vi "Stages Messenger.vi"(0 "Stage Notifier Name":string="ProScan3", 2 "Actions":T2, 5 "Setpoint":dbl[](array[numeric]), 7 "Axis":bool[](array[boolean]), 9 "Velocity":dbl, 11 "Misc":variant, 12 "Servo On?":bool, 13 "Exit While Busy?":bool) -> (4 "Stage Notifier Name (Dup)":string, 6 "Positions":dbl[](array[numeric]), 8 "Status":T1, 10 "Servo Status":bool, 15 "Error":errorcluster)   [LabVIEW 2021]
uses:
  Stages Controls/Stage Actions.ctl
  Stages Controls/Stage Status.ctl
  Stages Controls/Stage Notifier Element.ctl
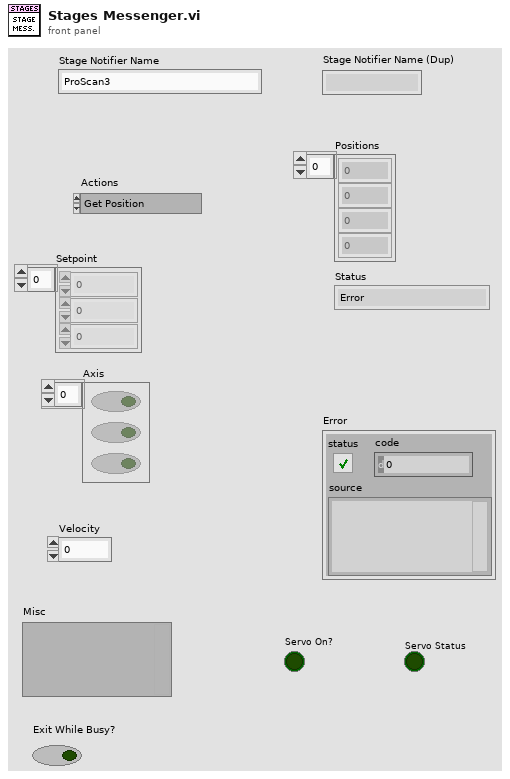
[diagram p1: front panel]
types:
  T1 = typedef "Stage Status.ctl" = enum16{"Error", "Abort", "Busy", "On Target"}
  T2 = typedef "Stage Actions.ctl" = enum16{"Get Position", "SERVO OFF", "SERVO ON", "SERVO ON/OFF", "MVR", "MOVE", "HALT", "ONTARGET", "ERROR", "REFERENCE", "INIT", "VELOCITY", "STATUS", "EXIT", "HOME", "ZEROPOS", "NANOPOS", "ANALOG", "QUIT"}
  T3 = typedef "Stage Notifier Element.ctl" = cluster{"Action":T2, "Axis":bool[], "Setpoint":dbl[], "Velocity":dbl, "Cmd Recvd?":bool, "Position":dbl[], "Status":T1, "Misc":variant, "Servo On?":bool}
  T4 = typedef "Stage Limits.ctl" = cluster{"Notifier":string, "Use Limits":bool, "Limits":dbl[][]}
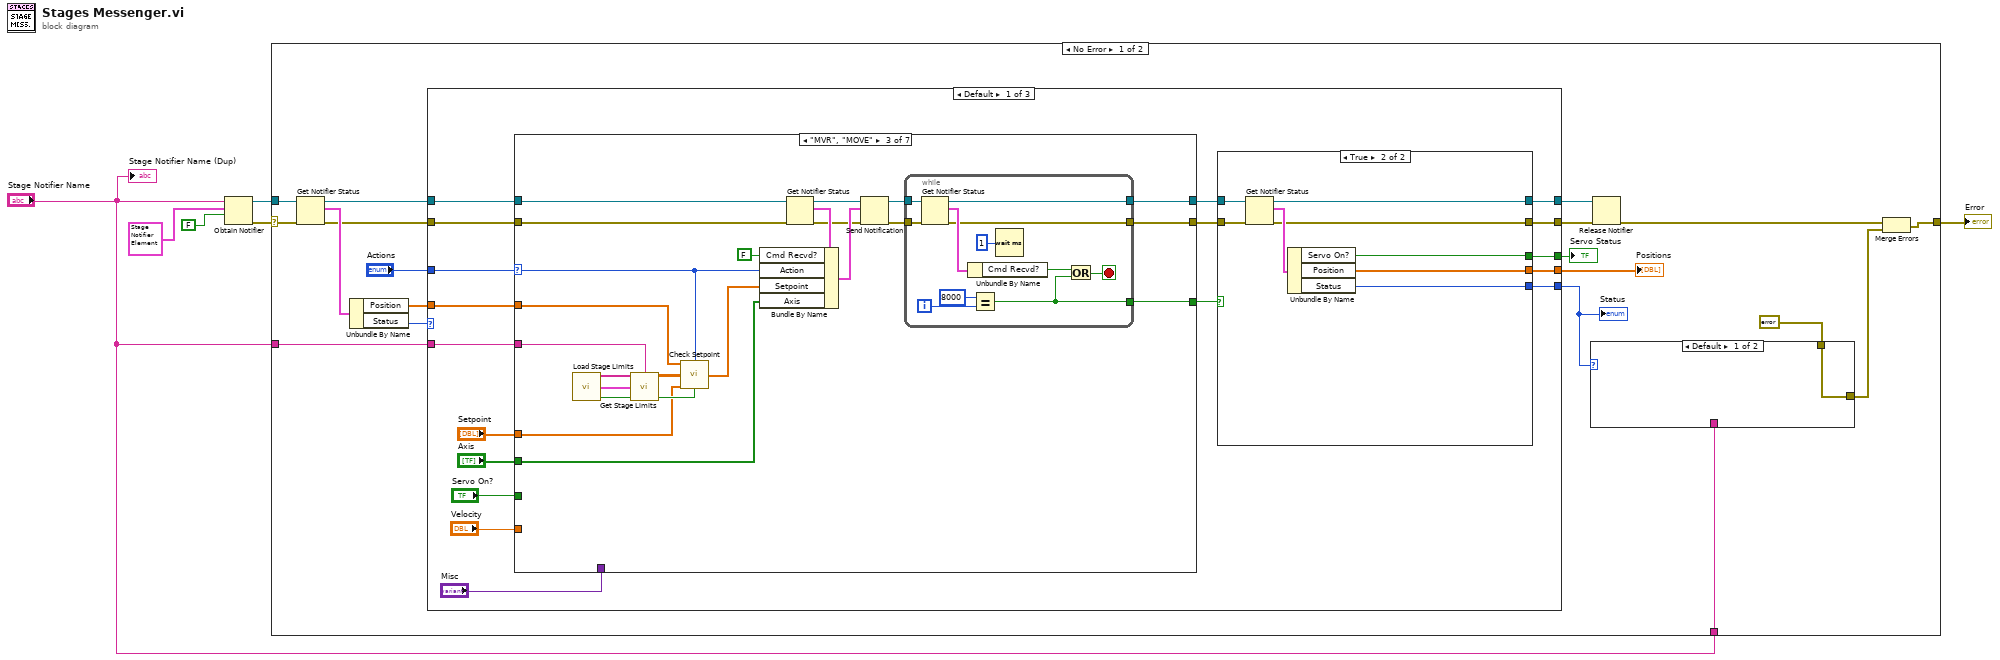
[diagram p0: block diagram]
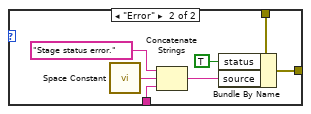
[diagram p2: hidden frame]
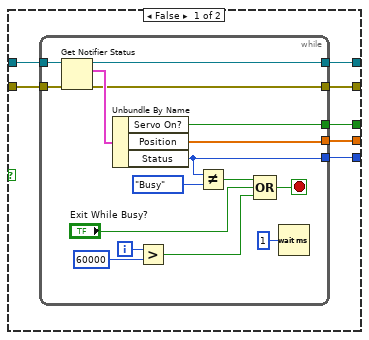
[diagram p3: hidden frame]
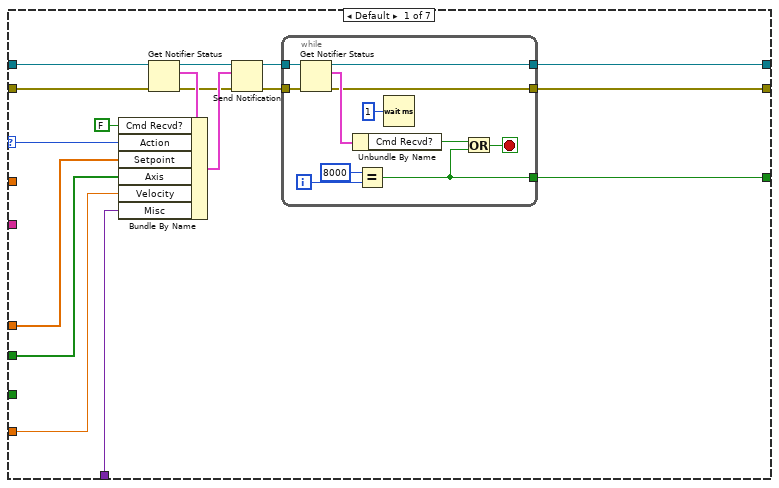
[diagram p4: hidden frame]
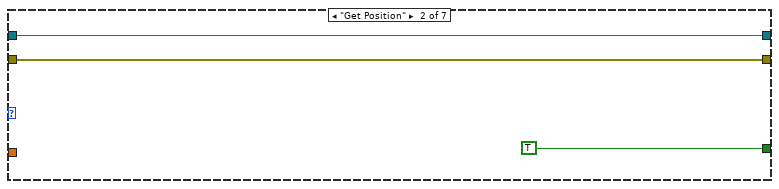
[diagram p5: hidden frame]
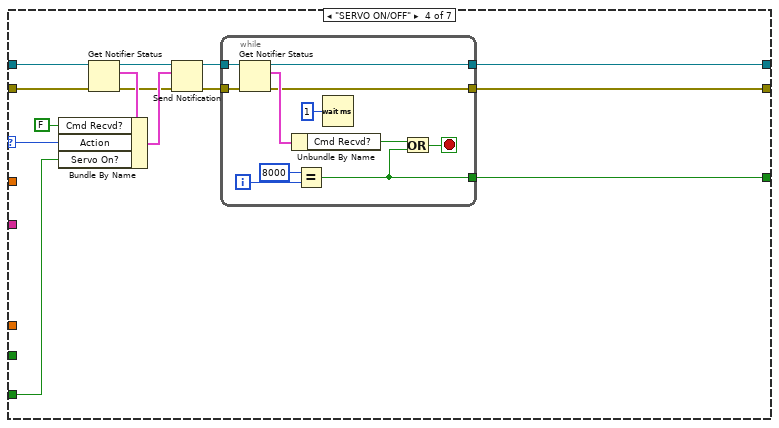
[diagram p6: hidden frame]
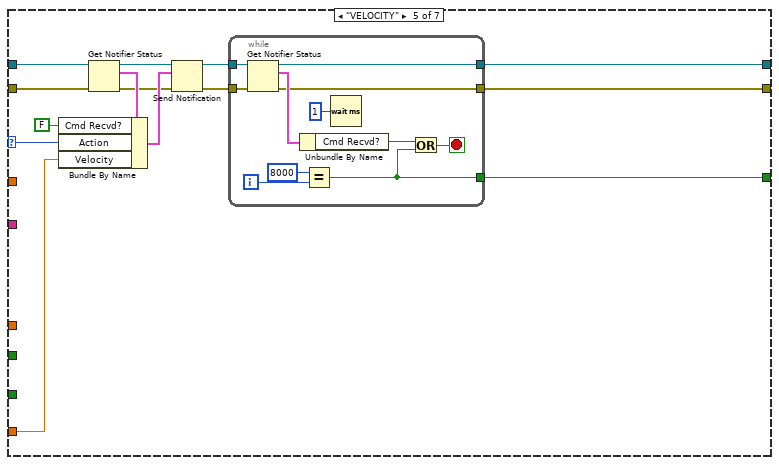
[diagram p7: hidden frame]
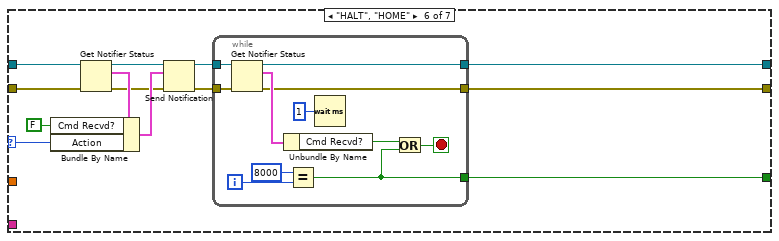
[diagram p8: hidden frame]
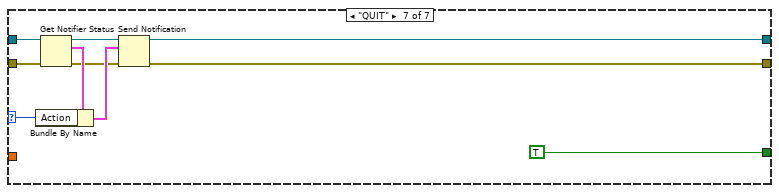
[diagram p9: hidden frame]
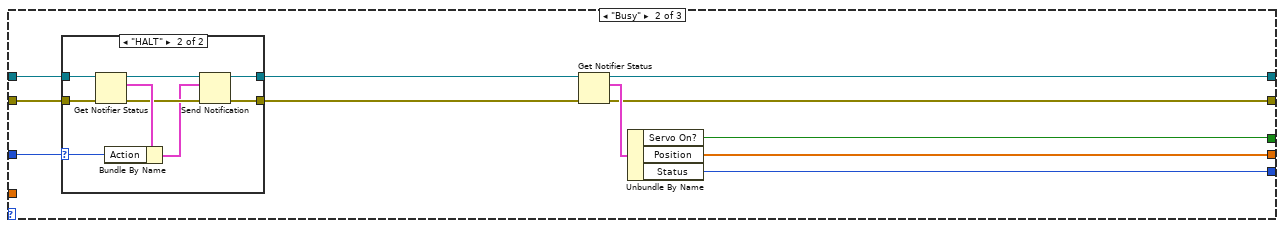
[diagram p10: hidden frame]
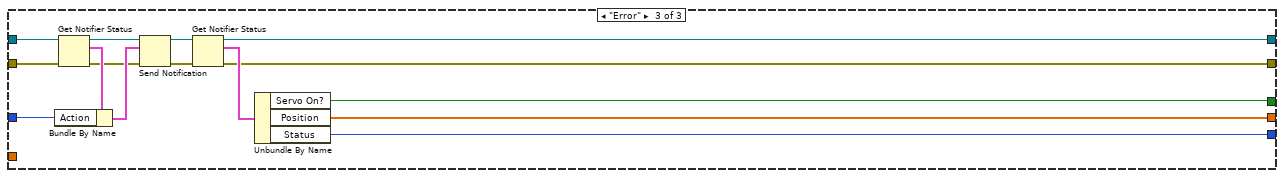
[diagram p12: hidden frame]
diagram:
  n1 = Obtain Notifier(name (unnamed)="Stage Notifier Name", notification data type=T3 {"Action"=enum."Get Position", "Axis"=[], "Setpoint"=[], "Velocity"=0.5, "Cmd Recvd?"=FALSE, "Position"=[], "Status"=enum."Error", "Misc"=variant, "Servo On?"=FALSE} ("Stage Status"), create if not found? (T)=FALSE) -> (notifier out=w3:refnum<notifier>, error out=w4:errorcluster)  [unwired: 1 in, 1 out]
  n2 = case shown="No Error" w4 {
    selector: w4 -> [w19 w269]
    tunnel: w3 -> [w25 _]
    tunnel: "Stage Notifier Name" -> [w14 _]
    tunnel: [w11 w269] -> w2
    tunnel: "Stage Notifier Name" -> [w7 _]
    frame No Error {
      n3 = Get Notifier Status(notifier=w25, error in (no error)=w19) -> (notifier out=w23:refnum<notifier>, current notification=w24:T3, error out=w18:errorcluster)  [unwired: 2 out]
      n4 = Unbundle By Name(w24) -> ("Position"=w8:dbl[], "Status"=w16:T1)
      n5 = case shown="Default" w16 {
        tunnel: w23 -> [w51 w236 w268]
        tunnel: [w44 w241 w262] -> w22
        tunnel: [w43 w240 w261] -> w21
        tunnel: [w42 w239 w260] -> w15
        tunnel: "Actions" -> [w50 w237 w266]
        tunnel: w18 -> [w41 w235 w258]
        tunnel: [w39 w238 w255] -> w17
        tunnel: [w36 w232 w254] -> w9
        tunnel: w8 -> [w35 _ _]
        tunnel: w7 -> [w34 _ _]
        frame Default {
          n6 = case shown="\"MVR\", \"MOVE\"" w50 {
            selector: w50 -> [w95 _ w119 w157 w182 w206 w227]
            tunnel: w51 -> [w96 w113 w133 w158 w183 w207 w230]
            tunnel: [w88 w113 w130 w154 w179 w203 w231] -> w45
            tunnel: "Setpoint" -> [w92 _ w116 _ _ _ _]
            tunnel: "Axis" -> [w91 _ w115 _ _ _ _]
            tunnel: "Velocity" -> [w90 _ _ _ w173 _ _]
            tunnel: "Misc" -> [w89 _ _ _ _ _ _]
            tunnel: [w87 TRUE w129 w153 w178 w202 TRUE] -> w46
            tunnel: w41 -> [w86 w112 w128 w152 w177 w201 w224]
            tunnel: [w83 w112 w125 w149 w174 w198 w222] -> w40
            tunnel: "Servo On?" -> [_ _ _ w148 _ _ _]
            tunnel: w35 -> [_ _ w118 _ _ _ _]
            tunnel: w34 -> [_ _ w117 _ _ _ _]
            frame Default {
              n7 = Get Notifier Status(notifier=w96, error in (no error)=w86) -> (notifier out=w97:refnum<notifier>, current notification=w98:T3, error out=w85:errorcluster)  [unwired: 2 out]
              n8 = Bundle By Name(cluster=w98, "Cmd Recvd?"=FALSE, "Action"=w95, "Setpoint"=w92, "Axis"=w91, "Velocity"=w90, "Misc"=w89) -> (w99:T3)
              n9 = Send Notification(notification=w99, notifier=w97, error in (no error)=w85) -> (notifier out=w93:refnum<notifier>, error out=w84:errorcluster)
              n10 = while {
                tunnel: w93 -> [w110]
                tunnel: [w107] -> w88
                tunnel: [w103] -> w87
                tunnel: w84 -> [w101]
                tunnel: [w100] -> w83
                i -> [w106]
                stop <- w102 stop-if-true
                n11 = Get Notifier Status(notifier=w110, error in (no error)=w101) -> (notifier out=w107:refnum<notifier>, current notification=w109:T3, error out=w100:errorcluster)  [unwired: 2 out]
                n12 = Unbundle By Name(w109) -> ("Cmd Recvd?"=w104:bool)
                n13 = Equal?(x=8000, y=w106) -> (x = y?=w103:bool)
                n14 = Wait (ms)(milliseconds to wait=u32 1) -> ()  [unwired: 1 out]
                n15 = Or(x=w104, y=w103) -> (x .or. y?=w102:bool)
              }
            }
            frame "Get Position" {
            }
            frame "MVR", "MOVE" {
              n16 = call "Load Stage Limits.vi"() -> ("Notifier Names"=w122:string[], "Stage Limits"=w123:T4[], "Loaded"=w124:bool)  [unwired: 13 in]
              n17 = call "Get Stage Limits.vi"("Notifier Names"=w122, "Notifier Name"=w117, "Stage Limits"=w123, "Limits Loaded?"=w124) -> ("Limits"=w120:dbl[][], "Use Limits?"=w121:bool)  [unwired: 10 in]
              n18 = call "Check Setpoint.vi"("Positions"=w118, "Actions"=w119, "Limits"=w120, "Setpoints"=w116, "Use Limits"=w121) -> ("Setpoints Out"=w114:dbl[])  [unwired: 10 in]
              n19 = Get Notifier Status(notifier=w133, error in (no error)=w128) -> (notifier out=w134:refnum<notifier>, current notification=w135:T3, error out=w127:errorcluster)  [unwired: 2 out]
              n20 = Bundle By Name(cluster=w135, "Cmd Recvd?"=FALSE, "Action"=w119, "Setpoint"=w114, "Axis"=w115) -> (w136:T3)
              n21 = Send Notification(notification=w136, notifier=w134, error in (no error)=w127) -> (notifier out=w131:refnum<notifier>, error out=w126:errorcluster)
              n22 = while {
                tunnel: w131 -> [w147]
                tunnel: [w144] -> w130
                tunnel: [w140] -> w129
                tunnel: w126 -> [w138]
                tunnel: [w137] -> w125
                i -> [w143]
                stop <- w139 stop-if-true
                n23 = Get Notifier Status(notifier=w147, error in (no error)=w138) -> (notifier out=w144:refnum<notifier>, current notification=w146:T3, error out=w137:errorcluster)  [unwired: 2 out]
                n24 = Unbundle By Name(w146) -> ("Cmd Recvd?"=w141:bool)
                n25 = Equal?(x=8000, y=w143) -> (x = y?=w140:bool)
                n26 = Wait (ms)(milliseconds to wait=u32 1) -> ()  [unwired: 1 out]
                n27 = Or(x=w141, y=w140) -> (x .or. y?=w139:bool)
              }
            }
            frame "SERVO ON/OFF" {
              n28 = Get Notifier Status(notifier=w158, error in (no error)=w152) -> (notifier out=w159:refnum<notifier>, current notification=w160:T3, error out=w151:errorcluster)  [unwired: 2 out]
              n29 = Bundle By Name(cluster=w160, "Cmd Recvd?"=FALSE, "Action"=w157, "Servo On?"=w148) -> (w161:T3)
              n30 = Send Notification(notification=w161, notifier=w159, error in (no error)=w151) -> (notifier out=w155:refnum<notifier>, error out=w150:errorcluster)
              n31 = while {
                tunnel: w155 -> [w172]
                tunnel: [w169] -> w154
                tunnel: [w165] -> w153
                tunnel: w150 -> [w163]
                tunnel: [w162] -> w149
                i -> [w168]
                stop <- w164 stop-if-true
                n32 = Get Notifier Status(notifier=w172, error in (no error)=w163) -> (notifier out=w169:refnum<notifier>, current notification=w171:T3, error out=w162:errorcluster)  [unwired: 2 out]
                n33 = Unbundle By Name(w171) -> ("Cmd Recvd?"=w166:bool)
                n34 = Equal?(x=8000, y=w168) -> (x = y?=w165:bool)
                n35 = Wait (ms)(milliseconds to wait=u32 1) -> ()  [unwired: 1 out]
                n36 = Or(x=w166, y=w165) -> (x .or. y?=w164:bool)
              }
            }
            frame "VELOCITY" {
              n37 = Get Notifier Status(notifier=w183, error in (no error)=w177) -> (notifier out=w184:refnum<notifier>, current notification=w185:T3, error out=w176:errorcluster)  [unwired: 2 out]
              n38 = Bundle By Name(cluster=w185, "Cmd Recvd?"=FALSE, "Action"=w182, "Velocity"=w173) -> (w186:T3)
              n39 = Send Notification(notification=w186, notifier=w184, error in (no error)=w176) -> (notifier out=w180:refnum<notifier>, error out=w175:errorcluster)
              n40 = while {
                tunnel: w180 -> [w197]
                tunnel: [w194] -> w179
                tunnel: [w190] -> w178
                tunnel: w175 -> [w188]
                tunnel: [w187] -> w174
                i -> [w193]
                stop <- w189 stop-if-true
                n41 = Get Notifier Status(notifier=w197, error in (no error)=w188) -> (notifier out=w194:refnum<notifier>, current notification=w196:T3, error out=w187:errorcluster)  [unwired: 2 out]
                n42 = Unbundle By Name(w196) -> ("Cmd Recvd?"=w191:bool)
                n43 = Equal?(x=8000, y=w193) -> (x = y?=w190:bool)
                n44 = Wait (ms)(milliseconds to wait=u32 1) -> ()  [unwired: 1 out]
                n45 = Or(x=w191, y=w190) -> (x .or. y?=w189:bool)
              }
            }
            frame "HALT", "HOME" {
              n46 = Get Notifier Status(notifier=w207, error in (no error)=w201) -> (notifier out=w208:refnum<notifier>, current notification=w209:T3, error out=w200:errorcluster)  [unwired: 2 out]
              n47 = Bundle By Name(cluster=w209, "Cmd Recvd?"=FALSE, "Action"=w206) -> (w210:T3)
              n48 = Send Notification(notification=w210, notifier=w208, error in (no error)=w200) -> (notifier out=w204:refnum<notifier>, error out=w199:errorcluster)
              n49 = while {
                tunnel: w204 -> [w221]
                tunnel: [w218] -> w203
                tunnel: [w214] -> w202
                tunnel: w199 -> [w212]
                tunnel: [w211] -> w198
                i -> [w217]
                stop <- w213 stop-if-true
                n50 = Get Notifier Status(notifier=w221, error in (no error)=w212) -> (notifier out=w218:refnum<notifier>, current notification=w220:T3, error out=w211:errorcluster)  [unwired: 2 out]
                n51 = Unbundle By Name(w220) -> ("Cmd Recvd?"=w215:bool)
                n52 = Equal?(x=8000, y=w217) -> (x = y?=w214:bool)
                n53 = Wait (ms)(milliseconds to wait=u32 1) -> ()  [unwired: 1 out]
                n54 = Or(x=w215, y=w214) -> (x .or. y?=w213:bool)
              }
            }
            frame "QUIT" {
              n55 = Get Notifier Status(notifier=w230, error in (no error)=w224) -> (notifier out=w229:refnum<notifier>, current notification=w228:T3, error out=w223:errorcluster)  [unwired: 2 out]
              n56 = Bundle By Name(cluster=w228, "Action"=w227) -> (w226:T3)
              n57 = Send Notification(notification=w226, notifier=w229, error in (no error)=w223) -> (notifier out=w231:refnum<notifier>, error out=w222:errorcluster)
            }
          }
          n58 = case shown="True" w46 {
            tunnel: w45 -> [w58 w82]
            tunnel: [w57 w81] -> w44
            tunnel: [w56 w80] -> w43
            tunnel: [w55 w78] -> w42
            tunnel: w40 -> [w54 w77]
            tunnel: [w53 w76] -> w39
            tunnel: [w52 w75] -> w36
            frame False {
              n59 = while {
                tunnel: w58 -> [w74]
                tunnel: [w73] -> w57
                tunnel: [w71] -> w56
                tunnel: [w65] -> w55
                tunnel: w54 -> [w61]
                tunnel: [w60] -> w53
                tunnel: [w59] -> w52
                i -> [w67]
                stop <- w62 stop-if-true
                n60 = Get Notifier Status(notifier=w74, error in (no error)=w61) -> (notifier out=w73:refnum<notifier>, current notification=w72:T3, error out=w60:errorcluster)  [unwired: 2 out]
                n61 = Unbundle By Name(w72) -> ("Servo On?"=w59:bool, "Position"=w71:dbl[], "Status"=w65:T1)
                n62 = Greater?(x=w67, y=60000) -> (0:w63:bool)
                n63 = Not Equal?(x=w65, y=Stage_Status."Busy") -> (x != y?=w68:bool)
                n64 = Compound Arithmetic op=OR(w68, "Exit While Busy?", w63) -> (w62:bool)
                n65 = Wait (ms)(milliseconds to wait=u32 1) -> ()  [unwired: 1 out]
              }
            }
            frame True {
              n66 = Get Notifier Status(notifier=w82, error in (no error)=w77) -> (notifier out=w81:refnum<notifier>, current notification=w79:T3, error out=w76:errorcluster)  [unwired: 2 out]
              n67 = Unbundle By Name(w79) -> ("Servo On?"=w75:bool, "Position"=w80:dbl[], "Status"=w78:T1)
            }
          }
        }
        frame "Busy" {
          n68 = case shown="\"HALT\"" w237 {
            selector: w237 -> [_ w250]
            tunnel: w236 -> [w244 w253]
            tunnel: w235 -> [w243 w252]
            tunnel: [w244 w247] -> w234
            tunnel: [w243 w246] -> w233
            frame Default {
            }
            frame "HALT" {
              n69 = Get Notifier Status(notifier=w253, error in (no error)=w252) -> (notifier out=w249:refnum<notifier>, current notification=w251:T3, error out=w248:errorcluster)  [unwired: 2 out]
              n70 = Bundle By Name(cluster=w251, "Action"=w250) -> (w245:T3)
              n71 = Send Notification(notification=w245, notifier=w249, error in (no error)=w248) -> (notifier out=w247:refnum<notifier>, error out=w246:errorcluster)
            }
          }
          n72 = Get Notifier Status(notifier=w234, error in (no error)=w233) -> (notifier out=w241:refnum<notifier>, current notification=w242:T3, error out=w238:errorcluster)  [unwired: 2 out]
          n73 = Unbundle By Name(w242) -> ("Servo On?"=w232:bool, "Position"=w240:dbl[], "Status"=w239:T1)
        }
        frame "Error" {
          n74 = Get Notifier Status(notifier=w268, error in (no error)=w258) -> (notifier out=w265:refnum<notifier>, current notification=w267:T3, error out=w257:errorcluster)  [unwired: 2 out]
          n75 = Bundle By Name(cluster=w267, "Action"=w266) -> (w264:T3)
          n76 = Send Notification(notification=w264, notifier=w265, error in (no error)=w257) -> (notifier out=w263:refnum<notifier>, error out=w256:errorcluster)
          n77 = Get Notifier Status(notifier=w263, error in (no error)=w256) -> (notifier out=w262:refnum<notifier>, current notification=w259:T3, error out=w255:errorcluster)  [unwired: 2 out]
          n78 = Unbundle By Name(w259) -> ("Servo On?"=w254:bool, "Position"=w261:dbl[], "Status"=w260:T1)
        }
      }
      "Positions" <- w21
      "Status" <- w15
      "Servo Status" <- w9
      n79 = case shown="Default" w15 {
        tunnel: w14 -> [_ w30]
        tunnel: [w26 w28] -> w12
        tunnel: errorcluster {"status"=FALSE, "code"=0, "source"=""} ("Error 2") -> [w26 w27]
        frame Default {
        }
        frame "Error" {
          n80 = call <vilib>:"Space Constant.vi"() -> ("String"=w31:string)
          n81 = Concatenate Strings("Stage status error." ("source"), w31, w30) -> (w29:string)
          n82 = Bundle By Name(cluster=w27, "status"=TRUE, "source"=w29) -> (w28:errorcluster)
        }
      }
      n83 = Release Notifier(notifier=w22, error in (no error)=w17) -> (error out=w13:errorcluster)  [unwired: 1 in, 2 out]
      n84 = Merge Errors(w13, w12) -> (w11:errorcluster)
    }
    frame Error {
    }
  }
  "Error" <- w2
  "Stage Notifier Name (Dup)" <- "Stage Notifier Name"
